vi "2LevelPassword.vi"(6 "password":string[](array[string])=["888888", "888666"], 11 "路径":path) -> (2 "Result":i32)   [LabVIEW 2025]
panel:
  in  "Title":string="请输入管理员或操作员密码\nPlease Input Administrator/Operator Password"
  in  "operator":bool
  in  "admin":bool
  in  "Exit":bool caption="Cancel"
  in  "pw":string
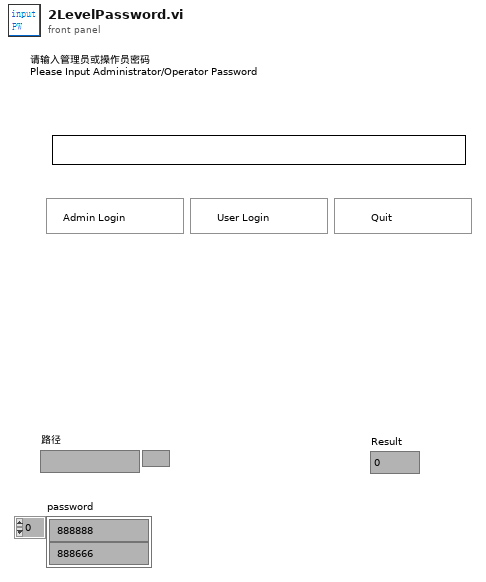
[diagram p1: front panel]
types:
  T1 = enum16{"open", "replace", "create", "open or create", "replace or create", "replace or create with confirmation"}
  T2 = enum32{"Invalid", "Standard", "Closed", "Hidden", "Minimized", "Maximized"}
  T3 = enum16{"ASCII", "Enter", "Return", "Shift", "Ctrl", "Alt", "Cmd", "Opt", "Caps", "NumLock", "Clear", "Break", "Up", "Down", "Left", "Right", "Insert", "Delete", "Home", "End", "PageUp", "PageDown", "Escape", "Help", "Pause", "ScrollLock", "F1", "F2", "F3", "F4", "F5", "F6", "F7", "F8", "F9", "F10", "F11", "F12", "F13", "F14", "F15", "F16", "F17", "F18", "F19", "F20", "F21", "F22", "F23", "F24", "Play", "VolumeUp", "VolumeDown", "Mute", "Two Byte Char"}
  T4 = typedef "eventvkey.ctl" = enum16{"ASCII", "Enter", "Return", "Shift", "Ctrl", "Alt", "Cmd", "Opt", "Caps", "NumLock", "Clear", "Break", "Up", "Down", "Left", "Right", "Insert", "Delete", "Home", "End", "PageUp", "PageDown", "Escape", "Help", "Pause", "ScrollLock", "F1", "F2", "F3", "F4", "F5", "F6", "F7", "F8", "F9", "F10", "F11", "F12", "F13", "F14", "F15", "F16", "F17", "F18", "F19", "F20", "F21", "F22", "F23", "F24", "Play", "VolumeUp", "VolumeDown", "Mute", "Two Byte Char"}
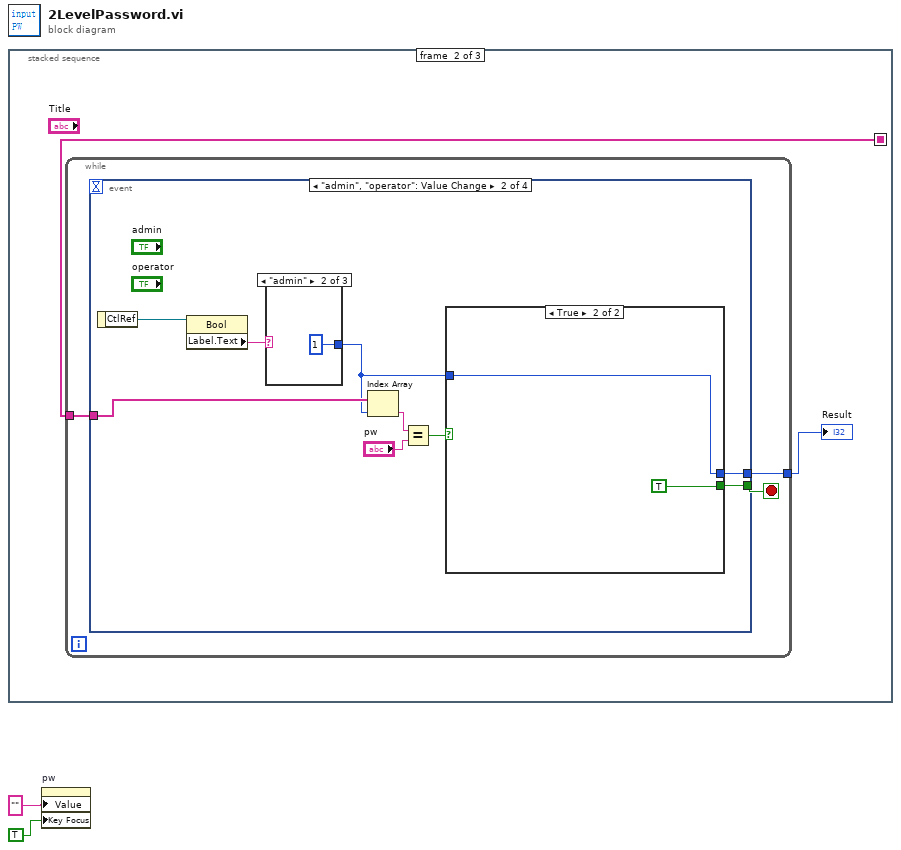
[diagram p0: block diagram]
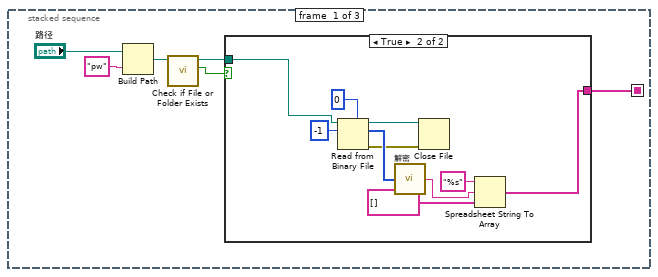
[diagram p2: hidden frame]
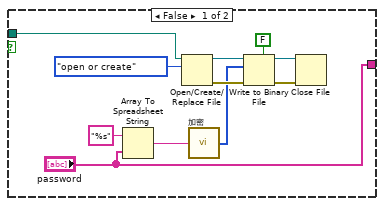
[diagram p3: hidden frame]
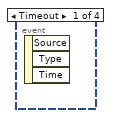
[diagram p4: hidden frame]
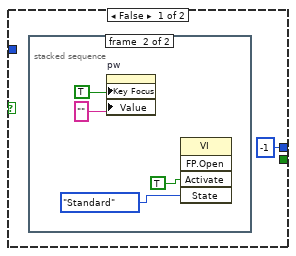
[diagram p5: hidden frame]
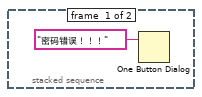
[diagram p6: hidden frame]
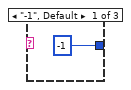
[diagram p7: hidden frame]
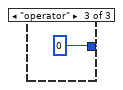
[diagram p8: hidden frame]
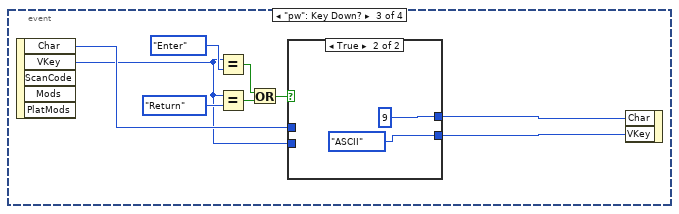
[diagram p9: hidden frame]
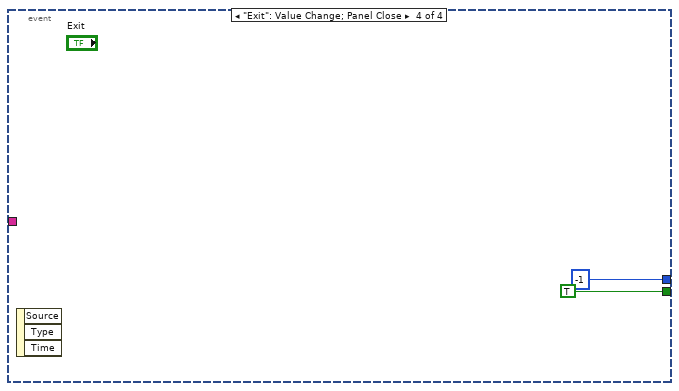
[diagram p11: hidden frame]
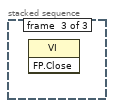
[diagram p12: hidden frame]
diagram:
  n1 = stacked-sequence {
    seq-local: [w5 _ _] -> [_ w31 _]
    frame #0 {
      n2 = Build Path(base path="路径", name or relative path="pw" ("名称或相对路径")) -> (appended path=w4:path)
      n3 = call <vilib>:"Check if File or Folder Exists.vi"("path"=w4) -> ("file or folder exists?"=w7:bool, "dup path"=w8:path)  [unwired: 8 in, 1 out]
      n4 = case shown="True" w7 {
        tunnel: w8 -> [w10 w22]
        tunnel: ["password" w20] -> w5
        frame False {
          n5 = Array To Spreadsheet String(array="password", 3:"%s" ("格式字符串")) -> (spreadsheet string=w14:string)  [unwired: 1 in]
          n6 = Open/Create/Replace File(file path (use dialog)=w10, operation (0:open)=T1."open or create" ("操作(0:open)")) -> (refnum out=w16:refnum<file>, error out=w19:errorcluster)  [unwired: 4 in, 1 out]
          n7 = call "加密.vi"("Text"=w14) -> ("Data"=w12:u8[])  [unwired: 4 in]
          n8 = Write to Binary File(file (use dialog)=w16, data=w12, error in=w19, 5:FALSE ("预置数组或字符串大小？(T)")) -> (refnum out=w11:refnum<file>, error out=w13:errorcluster)  [unwired: 2 in, 1 out]
          n9 = Close File(refnum=w11, error in=w13) -> ()  [unwired: 2 out]
        }
        frame True {
          n10 = Read from Binary File(5:u8 0, 10:-1 ("总数(1)"), 11:w22) -> (0:w21:errorcluster, 2:w27:u8[], 3:w25:refnum<file>)  [unwired: 3 in, 1 out]
          n11 = call "解密.vi"("Data"=w27) -> ("Text"=w28:string)  [unwired: 4 in]
          n12 = Close File(refnum=w25, error in=w21) -> ()  [unwired: 2 out]
          n13 = Spreadsheet String To Array(format string="%s" ("格式字符串"), spreadsheet string=w28, array type (2D Dbl)=string[] []) -> (array=w20:string[])  [unwired: 1 in]
        }
      }
    }
    frame #1 {
      n14 = while {
        tunnel: [w34] -> w30
        tunnel: w31 -> [w32]
        stop <- w33 stop-if-true
        n15 = event shown="[1] \"admin\", \"operator\": Value Change" {
          selector: _ -> [_ _ _ _]
          dyn-events: _ -> [_ _ _ _]
          timeout: _ -> [_ _ _ _]
          tunnel: [_ w36 _ -1 ("index of element")] -> w34
          tunnel: [_ w37 _ TRUE] -> w33
          tunnel: w32 -> [_ w41 _ _]
          event Timeout {
            n16 = event-data() -> ()  [unwired: 1 in, 3 out]
          }
          event "admin", "operator": Value Change {
            n17 = event-data() -> ("CtlRef"=w43:refnum<vi>)  [unwired: 1 in]
            n18 = property class="Bool"(reference=w43) -> ("Label.Text"=w42:string)  [unwired: 1 in, 2 out]
            n19 = case shown="\"admin\"" w42 {
              tunnel: [-1 1 0] -> w35
              frame "-1", Default {
              }
              frame "admin" {
              }
              frame "operator" {
              }
            }
            n20 = Index Array(array=w41, index=w35) -> (element=w40:string)
            n21 = Equal?(x=w40, y="pw") -> (x = y?=w38:bool)
            n22 = case shown="True" w38 {
              tunnel: [_ TRUE] -> w37
              tunnel: [-1 w50] -> w36
              tunnel: w35 -> [_ w50]
              frame False {
                n23 = stacked-sequence {
                  frame #0 {
                    n24 = One Button Dialog(message="密码错误！！！" ("消息")) -> ()  [unwired: 1 in, 1 out]
                  }
                  frame #1 {
                    n25 = property on="pw" class="Str"("Key Focus"=TRUE ("键选中"), "Value"="" ("pw")) -> ()  [unwired: 2 in, 2 out]
                    n26 = invoke class="VI" method="FP.Open"("Activate"=TRUE ("激活？"), "State"=T2."Standard" ("状态")) -> ()  [unwired: 3 in, 5 out]
                  }
                }
              }
              frame True {
              }
            }
          }
          event "pw": Key Down? {
            n27 = event-data() -> ("Char"=w57:i16, "VKey"=w55:T4)  [unwired: 1 in, 3 out]
            n28 = Equal?(x=w55, y=T3."Enter" ("V键")) -> (x = y?=w61:bool)
            n29 = Equal?(x=w55, y=T3."Return" ("V键")) -> (x = y?=w60:bool)
            n30 = Or(x=w61, y=w60) -> (x .or. y?=w59:bool)
            n31 = case shown="True" w59 {
              tunnel: [w65 i16 9 ("字符")] -> w58
              tunnel: w57 -> [w65 _]
              tunnel: [w64 T3."ASCII" ("VKey")] -> w56
              tunnel: w55 -> [w64 _]
              frame False {
              }
              frame True {
              }
            }
            n32 = event-data("Char"=w58, "VKey"=w56) -> ()  [unwired: 1 in, 1 out]
          }
          event "Exit": Value Change; Panel Close {
            n33 = event-data() -> ()  [unwired: 1 in, 3 out]
          }
        }
      }
      "Result" <- w30
    }
    frame #2 {
      n34 = invoke class="VI" method="FP.Close"() -> ()  [unwired: 3 in, 3 out]
    }
  }
  n35 = property on="pw" class="Str"("Value"="" ("pw"), "Key Focus"=TRUE ("键选中")) -> ()  [unwired: 2 in, 2 out]
